vi "PicoScope2000ExampleFastStreaming.vi"() -> ()   [LabVIEW 2010]
uses:
  ps2000.dll
  PicoScope2000Lib/PicoScope2000AnalogChannelSettings.ctl
panel:
  out "Channel A - Post capture raw data":T1(graph)
  out "Post capture information":T2
  out "Unit Info":T3
  out "overflow":i16 format="%02b"
  in  "Trigger Settings":T4={"Trigger Enabled"=FALSE, "Trigger Source"=enum."Channel A", "Trigger Threshold (V)"=0.0, "Trigger Direction"=0, "Trigger Delay (%)"=0, "Auto Trigger Time (ms)"=1000} {"Trigger Direction" items=["Rising", "Falling"]; "Trigger Threshold (V)" format="%.3f"}
  in  "Channel B Settings":T5={"Enabled"=FALSE, "Coupling"=1, "Range"=6} {"Range" items=["20 mV"=1, "50 mV"=2, "100 mV"=3, "200 mV"=4, "500 mV"=5, "1 V"=6, "2 V"=7, "5 V"=8, "10 V"=9, "20 V"=10]; "Coupling" items=["AC", "DC"]}
  in  "Channel A Settings":T5={"Enabled"=TRUE, "Coupling"=1, "Range"=6} {"Range" items=["20 mV"=1, "50 mV"=2, "100 mV"=3, "200 mV"=4, "500 mV"=5, "1 V"=6, "2 V"=7, "5 V"=8, "10 V"=9, "20 V"=10]; "Coupling" items=["AC", "DC"]}
  out "Raw Sample Interval (sec)":dbl=1.0000000130088963e-06 format="%#.5p"
  out "DownSample Interval (sec)":dbl=1.0000000130088963e-06 format="%#.5p"
  out "Previous Total":u32
  out "Number of Samples":u32
  out "Channel A - Live":i16[](graph)
  out "Total Samples":u32
  out "Auto Stopped":bool
  out "Application Buffer Full":bool
  out "Trigger":cluster{bool, "triggeredAt  Index (Total)":u32}
  in  "stop":bool
  in  "Acquisition Settings":T6={"Auto Stop"=TRUE, "Desired Sample Interval"=1, "Max Samples"=2000000, "Num Samples per Aggregate"=1, "Overview Buffer Size"=200000, "Time Units"=3, "Application Buffer Size"=25000000} {"Time Units" items=["Nanoseconds (ns)"=2, "Microseconds (us)"=3, "Milliseconds (ms)"=4, "Seconds (s)"=5]}
  # "It is now RECOMMENDED to use the newer PicoScope2000ExampleStreaming.vi example instead"
  # "NOTE: This chart is for indication purposes only - retrieve data values from the app buffer or driver post capture."
  # "Triggered"
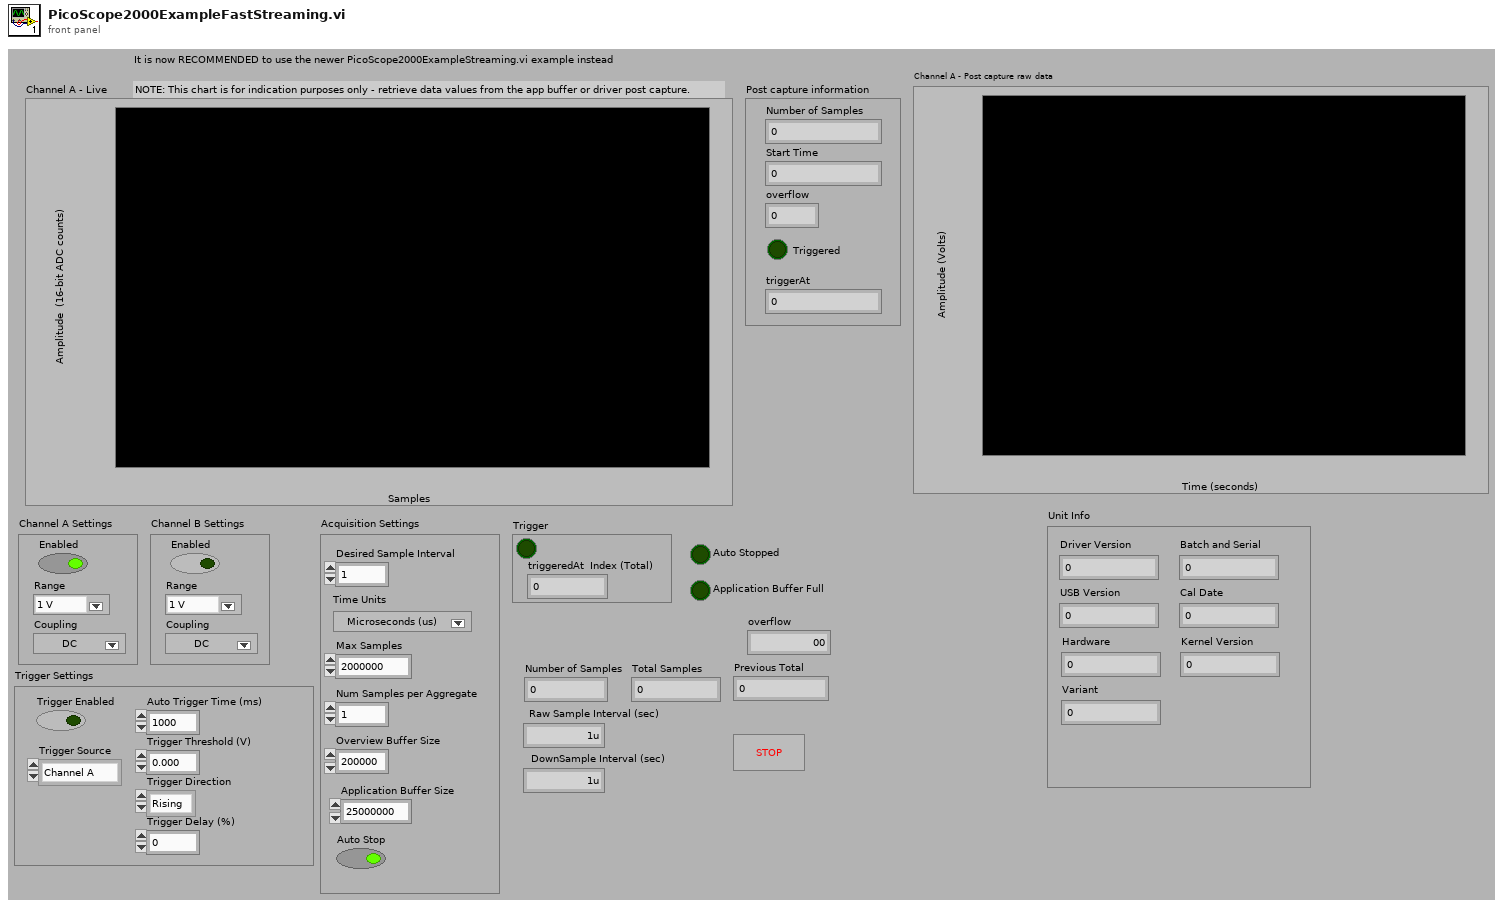
[diagram p1: front panel]
types:
  T1 = cluster{i32, "DownSample Interval (sec)":dbl, "Data":dbl[]}
  T2 = cluster{"Number of Samples":u32, "Start Time":dbl, "overflow":i16, bool, "triggerAt":u32}
  T3 = cluster{"Driver Version":string, "USB Version":string, "Hardware":string, "Variant":string, "Batch and Serial":string, "Cal Date":string, "Kernel Version":string}
  T4 = cluster{"Trigger Enabled":bool, "Trigger Source":enum16{"Channel A", "Channel B", "Channel C", "Channel D", "Ext."}, "Trigger Threshold (V)":dbl, "Trigger Direction":i16, "Trigger Delay (%)":i16, "Auto Trigger Time (ms)":i16}
  T5 = typedef "PicoScope2000AnalogChannelSettings.ctl" = cluster{"Enabled":bool, "Coupling":i16, "Range":u16}
  T6 = cluster{"Auto Stop":bool, "Desired Sample Interval":u32, "Max Samples":u32, "Num Samples per Aggregate":u32, "Overview Buffer Size":u32, "Time Units":u32, "Application Buffer Size":u32}
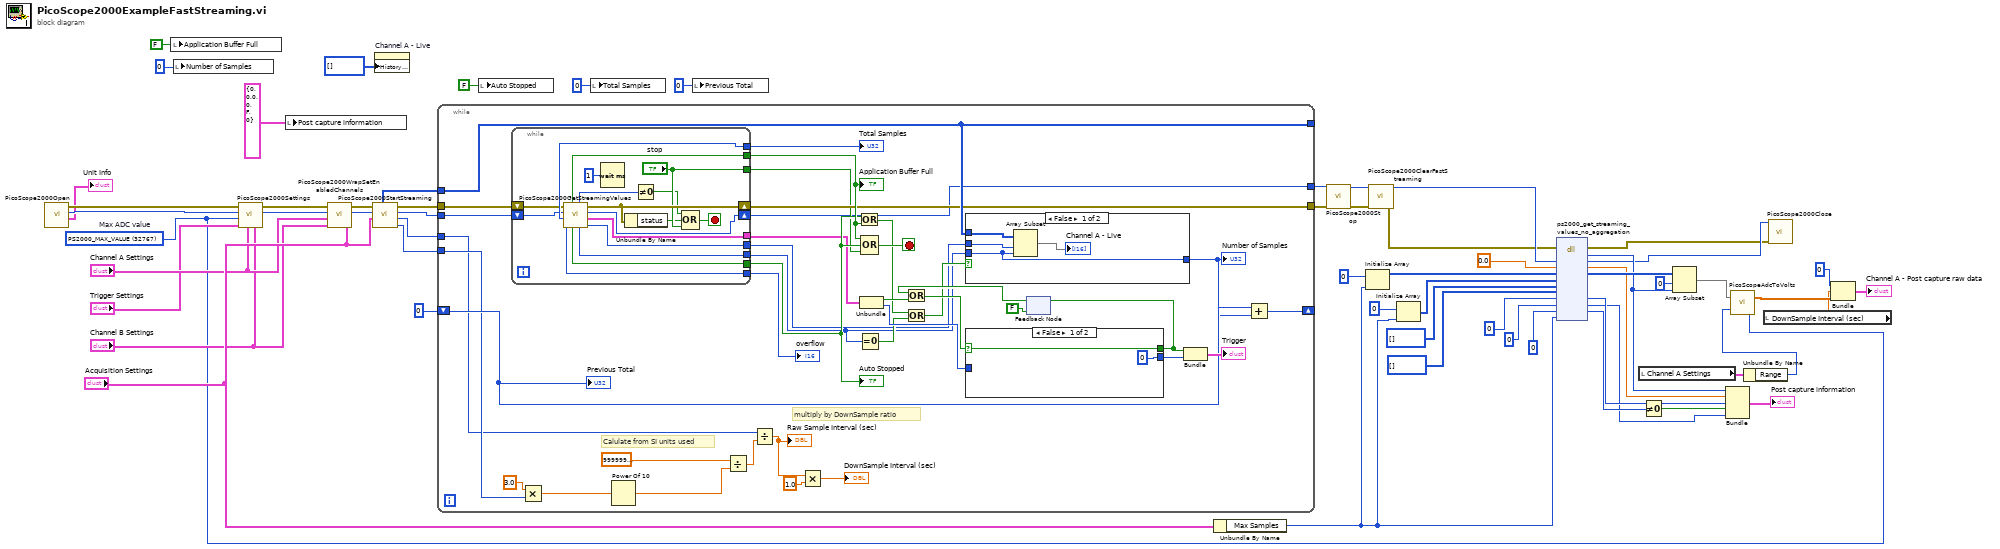
[diagram p0: block diagram]
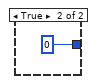
[diagram p2: hidden frame]
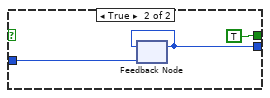
[diagram p3: hidden frame]
diagram:
  w10 = i16 32767 items=["PS2000_MAX_VALUE"=32767]  # Max ADC value
  n1 = call "PicoScope2000Open.vi"() -> ("Unit Info"=→"Unit Info":T3, "handle"=w59:i16, "error out"=w60:errorcluster)  [unwired: 7 in]
  n2 = local write "Application Buffer Full"(FALSE ("Application Buffer Full")) -> ()
  n3 = local write "Number of Samples"(u32 0 ("Number of Samples")) -> ()
  n4 = call "PicoScope2000Settings.vi"("Channel B Settings"="Channel B Settings", "Channel A Settings"="Channel A Settings", "Trigger Settings"="Trigger Settings", "Max ADC value"=w10, "handle in"=w59, "error in"=w60) -> ("handle out"=w46:i16, "error out"=w58:errorcluster)  [unwired: 1 in, 1 out]
  n5 = local write "Post capture information"(T2 {"Number of Samples"=0, "Start Time"=0.0, "overflow"=0, FALSE, "triggerAt"=0} ("Post capture information")) -> ()
  n6 = call "PicoScope2000WrapSetEnabledChannels.vi"("Acquisition Settings"="Acquisition Settings", "Channel B Settings"="Channel B Settings", "Channel A Settings"="Channel A Settings", "handle in"=w46, "error in (no error)"=w58) -> ("handle out"=w45:i16, "error out"=w57:errorcluster)  [unwired: 1 in]
  n7 = call "PicoScope2000StartStreaming.vi"("Acquisition Settings"="Acquisition Settings", "handle in"=w45, "error in"=w57) -> ("time_units"=w43:u32, "Sample Interval"=w42:u32, "handle out"=w55:i16, "error out"=w56:errorcluster, "Channel A"=w54:i16[])  [unwired: 1 in, 1 out]
  n8 = property on="Channel A - Live" class="WFChart (strict)"("History Data"=i16[] []) -> ()  [unwired: 2 in, 2 out]
  n9 = while {
    tunnel: w56 -> [w66]
    tunnel: w55 -> [w65]
    tunnel: w54 -> [w83]
    tunnel: [w62] -> w4
    tunnel: [w64] -> w5
    shift-right: [w89] -> _
    shift-left: u32 0 -> [w88]
    tunnel: [w83] -> _
    tunnel: w43 -> [w75]
    tunnel: w42 -> [w74]
    stop <- w98 stop-if-true
    # "Calulate from SI units used"
    # "multiply by DownSample ratio"
    n10 = while {
      tunnel: [w115] -> w73
      tunnel: [w114] -> w72
      tunnel: [w113] -> w71
      tunnel: [w112] -> w70
      tunnel: [w111] -> w69
      tunnel: [w110] -> w68
      tunnel: [w109] -> w67
      shift-right: [w106] -> w64
      shift-left: w66 -> [w108]
      tunnel: ["stop"] -> w63
      shift-right: [w102] -> w62
      shift-left: w65 -> [w107]
      stop <- w105 stop-if-true
      n11 = call "PicoScope2000GetStreamingValues.vi"("handle in"=w107, "error in"=w108) -> ("App Buffer startIndex"=w111:u32, "Trigger"=w109:cluster{bool, "triggeredAt  Index (Total)":u32}, "handle out"=w102:i16, "error out"=w106:errorcluster, "Number of Samples"=w110:u32, "ready"=w101:i16, "Auto Stopped"=w113:bool, "Application Buffer Full"=w114:bool, "overflow"=w115:i16, "Total Samples"=w112:u32)
      n12 = Wait (ms)(milliseconds to wait=u32 1) -> ()  [unwired: 1 out]
      n13 = Unbundle By Name(w106) -> ("status"=w99:bool)
      n14 = Not Equal To 0?(x=w101) -> (x != 0?=w103:bool)
      n15 = Compound Arithmetic op=OR(w103, w99, "stop") -> (w105:bool)
    }
    "Application Buffer Full" <- w72
    "Auto Stopped" <- w71
    "Total Samples" <- w70
    "overflow" <- w73
    n16 = Multiply(x=3.0, y=w75) -> (x*y=w78:dbl)
    n17 = Power Of 10(x=w78) -> (10^x=w79:dbl)
    n18 = Divide(x=sgl 1000000000000000.0 ("y"), y=w79) -> (x/y=w80:dbl)
    n19 = Divide(x=w74, y=w80) -> (x/y=w77:dbl)
    "Raw Sample Interval (sec)" <- w77
    n20 = Multiply(x=w77, y=1.0) -> (x*y=→"DownSample Interval (sec)":dbl)
    n21 = Or(x=w71, y=w72) -> (x .or. y?=w86:bool)
    n22 = Equal To 0?(x=w68) -> (x = 0?=w84:bool)
    n23 = Unbundle(w67) -> (w91:bool, "triggeredAt  Index (Total)"=w96:u32)
    n24 = Compound Arithmetic op=OR(w72, w71, w63) -> (w98:bool)
    n25 = Or(x=w86, y=w84) -> (x .or. y?=w85:bool)
    n26 = case shown="False" w85 {
      tunnel: w69 -> [w119 _]
      tunnel: w83 -> [w118 _]
      tunnel: w68 -> [w117 _]
      tunnel: [w117 u32 0 ("Number of Samples")] -> w87
      frame False {
        n27 = Array Subset(array=w118, index=w119, length=w117) -> (→"Channel A - Live":i16[])
      }
      frame True {
      }
    }
    "Number of Samples" <- w87
    n28 = feedback #1(FALSE) -> (w92:bool)
    n29 = Or(x=w92, y=w91) -> (x .or. y?=w93:bool)
    n30 = case shown="False" w93 {
      selector: w93 -> [w122 _]
      tunnel: w96 -> [_ w125]
      tunnel: [u32 0 ("triggeredAt  Index (Total)") w124] -> w95
      tunnel: [w122 TRUE] -> w94
      frame False {
      }
      frame True {
        n31 = feedback #2(w125) -> (w124:u32)
        n32 = feedback-in #2(w124) -> ()
      }
    }
    n33 = feedback-in #1(w94) -> ()
    n34 = Bundle(w94, "triggeredAt  Index (Total)"=w95) -> (→"Trigger":cluster{bool, "triggeredAt  Index (Total)":u32})  [unwired: 1 in]
    n35 = Add(x=w88, y=w87) -> (x+y=w89:u32)
    "Previous Total" <- w88
  }
  n36 = local write "Auto Stopped"(FALSE ("Auto Stopped")) -> ()
  n37 = local write "Total Samples"(u32 0 ("Total Samples")) -> ()
  n38 = local write "Previous Total"(u32 0 ("Previous Total")) -> ()
  n39 = Unbundle By Name("Acquisition Settings") -> ("Max Samples"=w13:u32)
  n40 = call "PicoScope2000Stop.vi"("error in (no error)"=w5, "handle in"=w4) -> ("error out"=w9:errorcluster, "handle out"=w8:i16)  [unwired: 8 in]
  n41 = Initialize Array(i16 0 ("triggerAt"), w13) -> (w34:i16[])
  n42 = call "PicoScope2000ClearFastStreaming.vi"("error in"=w9, "handle"=w8) -> ("error out"=w6:errorcluster, "handle out"=w7:i16)  [unwired: 4 in]
  n43 = Initialize Array(i16 0 ("triggerAt"), w13) -> (w31:i16[])
  n44 = dll-call lib="ps2000.dll" fn="ps2000_get_streaming_values_no_aggregation"(error in=w6, "handle"=w7, "Start Time"=0.0 ("start_time"), "buffer_a"=w34, "buffer_b"=w31, "buffer_c"=i16[] [], "buffer_d"=i16[] [] ("buffer_c"), "overflow"=i16 0 ("triggerAt"), "triggerAt"=u32 0 ("number"), "trigger"=i16 0, "no_of_values"=w13) -> (error out=w15:errorcluster, "Number of Samples"=w28:u32, "handle"=w16:i16, "Start Time"=w27:dbl, "buffer_a"=w30:i16[], "overflow"=w25:i16, "triggerAt"=w23:u32, "trigger"=w26:i16)  [unwired: 6 in, 1 out]
  n45 = local read "Channel A Settings"() -> (w11:T5)
  n46 = Not Equal To 0?(x=w26) -> (x != 0?=w24:bool)
  n47 = Array Subset(array=w30, index=0, length=w28) -> (w17:i16[])
  n48 = Bundle("Number of Samples"=w28, "Start Time"=w27, "overflow"=w25, w24, "triggerAt"=w23) -> (→"Post capture information":T2)  [unwired: 1 in]
  n49 = Unbundle By Name(w11) -> ("Range"=w12:u16)
  n50 = call "PicoScopeAdcToVolts.vi"("Max_adc"=w10, "Range Index"=w12, "Data"=w17) -> ("Data"=w18:dbl[])
  n51 = local read "DownSample Interval (sec)"() -> (w3:dbl)
  n52 = call "PicoScope2000Close.vi"("error in"=w15, "handle"=w16) -> ()  [unwired: 4 in, 2 out]
  n53 = Bundle(0, "DownSample Interval (sec)"=w3, "Data"=w18) -> (→"Channel A - Post capture raw data":T1)  [unwired: 1 in]
